vi "2D Gaussian - Fit Image DBL.vi"(7 "Image In (DBL)":dbl[][](array[numeric]), 11 "Error In":errorcluster) -> (8 "Best Fit Params":T1, 15 "Error Out":errorcluster)   [LabVIEW 2016]
uses:
  2D Gaussian - Type Defs/2D Gaussian - Best Fit Parameters.ctl
  <vilib>/gmath/NumericalOptimization/Nonlinear Curve Fit LM bound.vi
  <vilib>/gmath/NI_Gmath.lvlib
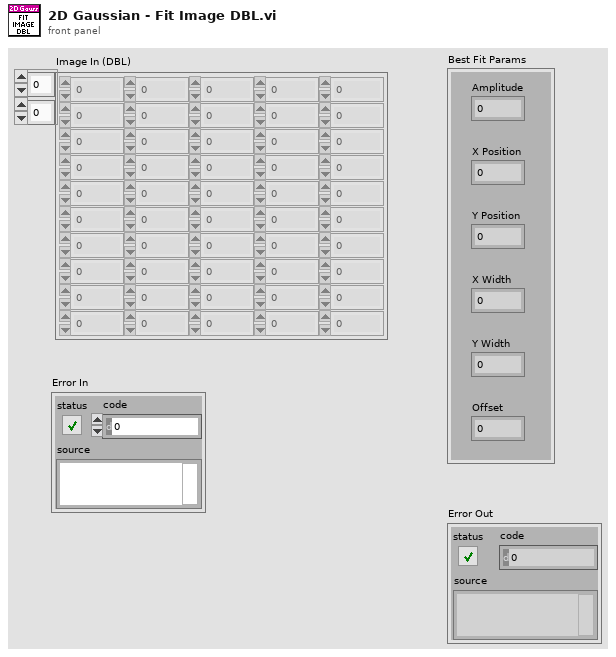
[diagram p1: front panel]
types:
  T1 = typedef "2D Gaussian - Best Fit Parameters.ctl" = cluster{"Amplitude":dbl, "X Position":dbl, "Y Position":dbl, "X Width":dbl, "Y Width":dbl, "Offset":dbl}
  T2 = cluster{"parameter minimum":dbl[], "parameter maximum":dbl[]}
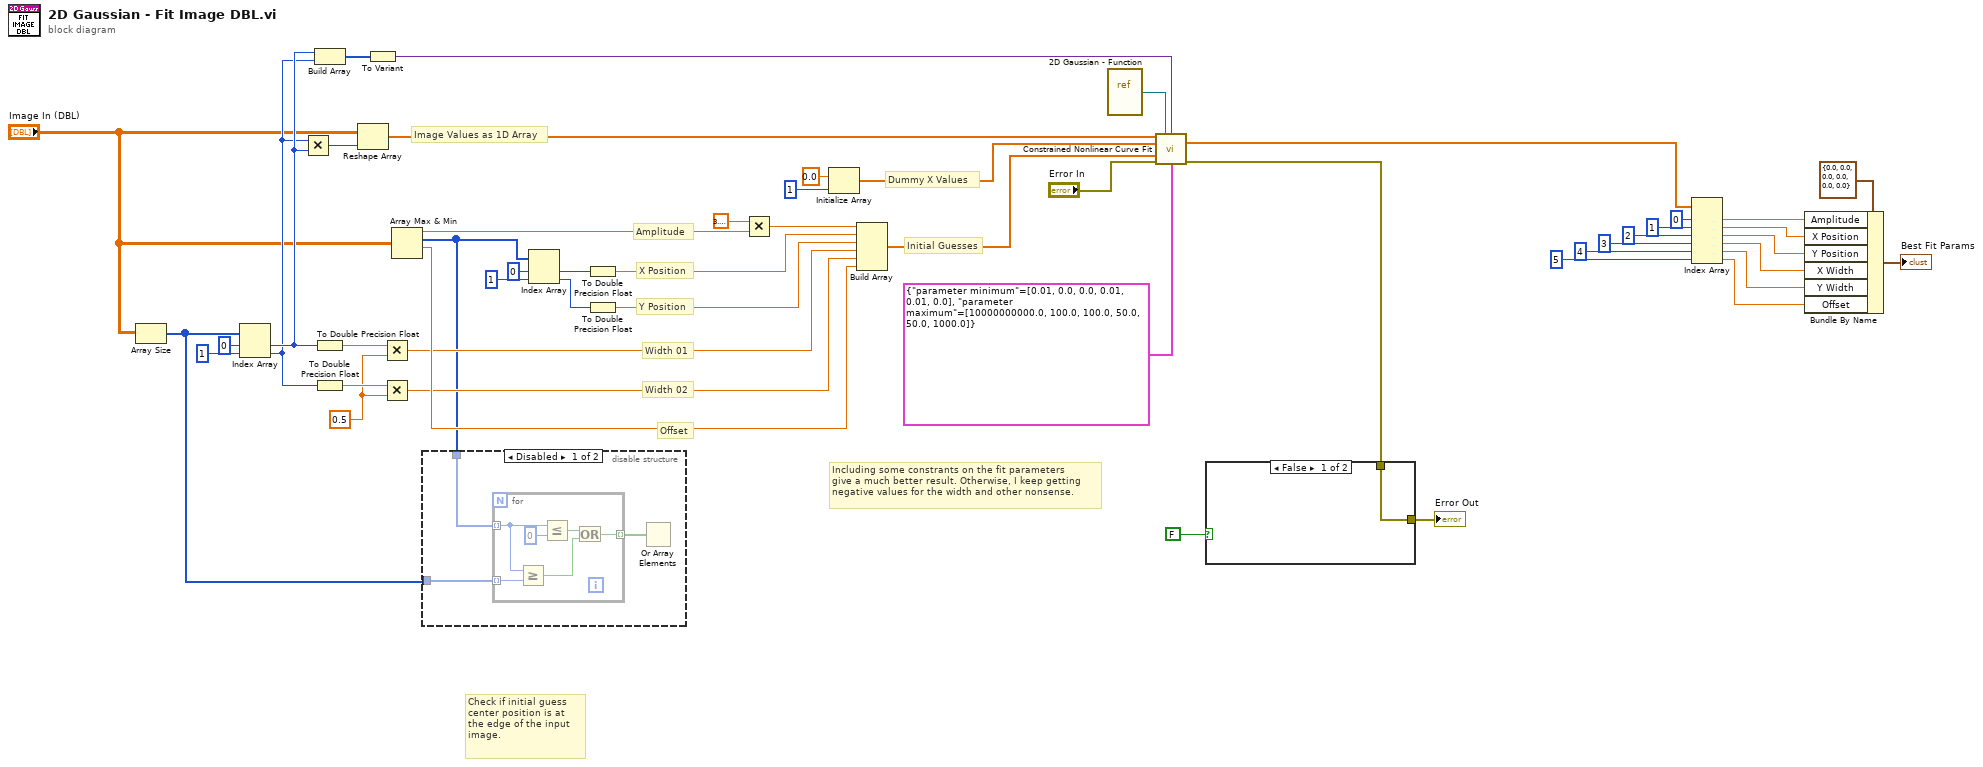
[diagram p0: block diagram]
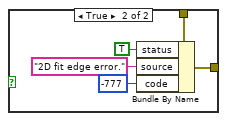
[diagram p3: hidden frame]
diagram:
  w36 = 0.5
  # "Check if initial guess center position is at the edge of the input image."
  # "Including some constrants on the fit parameters\ngive a much better result. Otherwise, I keep getting\nnegative values for the width and other nonsense."
  # "Dummy X Values"
  # "Image Values as 1D Array"
  # "Initial Guesses"
  # "Width 02"
  # "Width 01"
  # "Y Position"
  # "X Position"
  # "Offset"
  # "Amplitude"
  n1 = Array Size(array="Image In (DBL)") -> (size(s)=w3:i32[])
  n2 = Index Array(array=w3, index #1=0 ("index"), index #2=1 ("index")) -> (element #1=w27:i32, element #2=w26:i32)
  n3 = Multiply(x=w26, y=w27) -> (x*y=w32:i32)
  n4 = Build Array(w27, w26) -> (w25:i32[])
  n5 = To Double Precision Float(number=w27) -> (double precision float=w38:dbl)
  n6 = To Double Precision Float(number=w26) -> (double precision float=w37:dbl)
  n7 = Reshape Array("Image In (DBL)", w32) -> (w33:dbl[])
  n8 = To Variant(anything=w25) -> (Variant=w24:variant)
  n9 = Multiply(x=w38, y=w36) -> (x*y=w35:dbl)
  n10 = Multiply(x=w37, y=w36) -> (x*y=w34:dbl)
  n11 = Array Max & Min(array="Image In (DBL)") -> (max value=w49:dbl, max index (indices)=w4:i32[], min value=w47:dbl)  [unwired: 1 out]
  n12 = disable-structure shown="Disabled" {
    disable-tunnel: w4 -> [w54 _]
    disable-tunnel: w3 -> [w53 _]
    frame Disabled {
      n13 = for {
        tunnel: w54 -> [w59] mode=indexing
        tunnel: w53 -> [w60] mode=indexing
        tunnel: [w55] -> w52 mode=indexing
        n14 = Greater Or Equal?(x=w59, y=w60) -> (x >= y?=w56:bool)
        n15 = Less Or Equal?(x=w59, y=0) -> (x <= y?=w57:bool)
        n16 = Or(x=w57, y=w56) -> (x .or. y?=w55:bool)
      }
      n17 = Or Array Elements(Boolean array=w52) -> ()  [unwired: 1 out]
    }
    frame Enabled {
    }
  }
  n18 = Index Array(array=w4, index #1=0 ("index"), index #2=1 ("index")) -> (element #1=w44:i32, element #2=w42:i32)
  n19 = To Double Precision Float(number=w44) -> (double precision float=w43:dbl)
  n20 = To Double Precision Float(number=w42) -> (double precision float=w41:dbl)
  n21 = Multiply(x=3.141592653589793, y=w49) -> (x*y=w48:dbl)
  n22 = Initialize Array(0.0 ("element"), 1 ("dimension size")) -> (w30:dbl[])
  n23 = Build Array(w48, w43, w41, w35, w34, w47) -> (w29:dbl[])
  n24 = vi-ref "2D Gaussian - Function.vi"() -> (w51:refnum<vi>)
  n25 = call-poly <vilib>:"Constrained Nonlinear Curve Fit.vi"("Y"=w33, "f(x,a)"=w51, "data"=w24, "X"=w30, "initial parameters"=w29, "error in (no error)"="Error In", "parameter bounds"=T2 {"parameter minimum"=[0.01, 0.0, 0.0, 0.01, 0.01, 0.0], "parameter maximum"=[10000000000.0, 100.0, 100.0, 50.0, 50.0, 1000.0]}) -> ("best fit parameters"=w22:dbl[], "error out"=w5:errorcluster)  [unwired: 3 in, 4 out]
  n26 = case shown="False" FALSE {
    tunnel: w5 -> [w61 w66]
    tunnel: [w61 w62] -> w2
    frame False {
    }
    frame True {
      n27 = Bundle By Name(cluster=w66, "status"=TRUE, "source"="2D fit edge error.", "code"=-777) -> (w62:errorcluster)
    }
  }
  "Error Out" <- w2
  n28 = Index Array(array=w22, index #1=0 ("index"), index #2=1 ("index"), index #3=2 ("index"), index #4=3 ("index"), index #5=4 ("index"), index #6=5 ("index")) -> (element #1=w21:dbl, element #2=w20:dbl, element #3=w19:dbl, element #4=w18:dbl, element #5=w17:dbl, element #6=w16:dbl)
  n29 = Bundle By Name(cluster=T1 {"Amplitude"=0.0, "X Position"=0.0, "Y Position"=0.0, "X Width"=0.0, "Y Width"=0.0, "Offset"=0.0} ("Best Fit Parameters"), "Amplitude"=w21, "X Position"=w20, "Y Position"=w19, "X Width"=w18, "Y Width"=w17, "Offset"=w16) -> (→"Best Fit Params":T1)
